vi "test_DiscoveryServiceNotRunning_LaunchDiscoveryService_DiscoveryServiceStarted.vi"(8 "error in":errorcluster) -> (0 "error out":errorcluster, 2 "result":string, 3 "pass":bool)   [LabVIEW 2021, in "MeasurementServerTests.lvlib" / "Discovery Tests.lvlib"]
uses:
  Discovery Tests.lvlib
  Runtime/Clients/Discovery V1/TypeDefs/gRPC Client Cache FGV Action.ctl
  MeasurementServerTests.lvlib
  Runtime/Clients/Discovery V1/NI Discovery V1 Client.lvlib
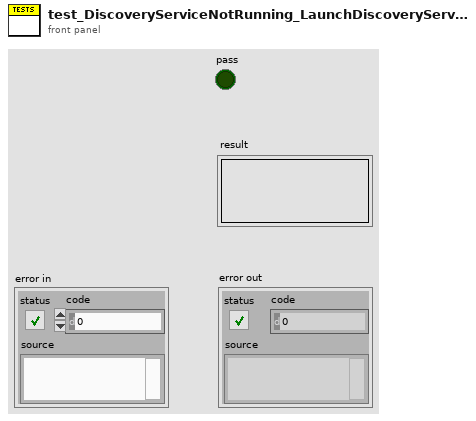
[diagram p1: front panel]
types:
  T1 = typedef "NI Discovery V1 Client.lvlib/gRPC Client Cache FGV Action.ctl" = enum16{"Get Client", "Recreate Client", "Destroy Client", "Update ClusterId"}
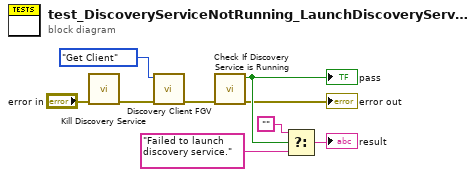
[diagram p0: block diagram]
diagram:
  n1 = call "Kill Discovery Service.vi"("error in"="error in") -> ("error out"=w3:errorcluster)  [unwired: 10 in]
  n2 = call "Discovery Client FGV.vi"("error in"=w3, "action"=gRPC_Client_Cache_FGV_Action."Get Client") -> ("error out"=w2:errorcluster)  [unwired: 6 in, 3 out]
  n3 = call "Check If Discovery Service is Running.vi"("error in"=w2) -> ("error out"=→"error out":errorcluster, "discovery service running?"=w5:bool)  [unwired: 9 in]
  "pass" <- w5
  n4 = Select(t="", s=w5, f="Failed to launch discovery service.") -> (s? t:f=→"result":string)
